vi "PeriodicFilter-Format Stop Filter Entrys.vi"(7 "Seconds Since 1Jan1904 2":timestamp, 10 "Time Format String":string="%<%H:%M:%S%3u>T", 11 "Removed Info":T1[](array[typedef])) -> (3 "Array":string[](array[string]))   [LabVIEW 2017, in "Communicable State Machine.lvlib"]
uses:
  Communicable State Machine.lvlib
  Periodic String Filter Info.ctl
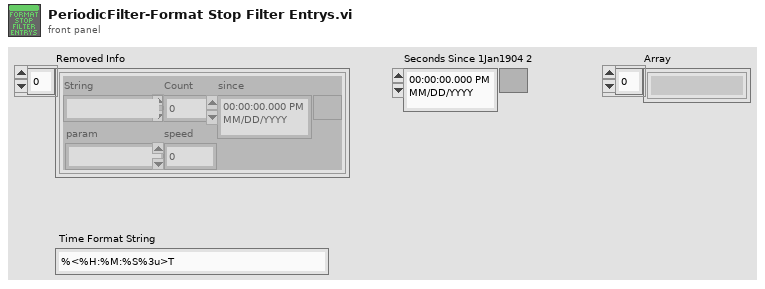
[diagram p1: front panel]
types:
  T1 = typedef "Communicable State Machine.lvlib/Periodic String Filter Info.ctl" = cluster{"String":string, "Count":i64, "since":timestamp, "param":string, "speed":dbl}
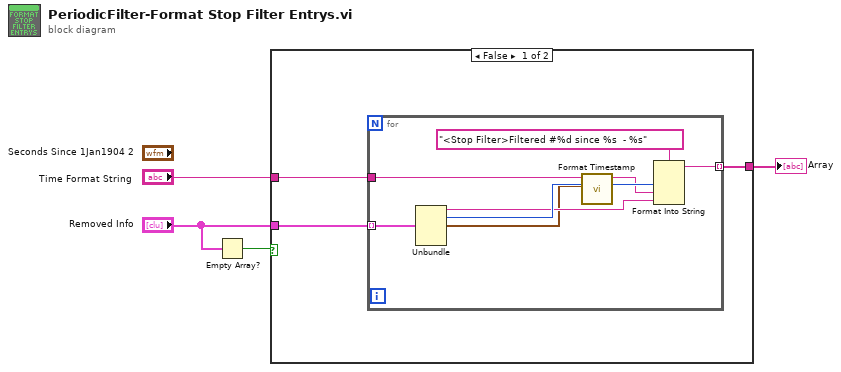
[diagram p0: block diagram]
diagram:
  n1 = Empty Array?(array="Removed Info") -> (empty?=w1:bool)
  n2 = case shown="False" w1 {
    tunnel: "Time Format String" -> [w7 _]
    tunnel: [w6 _] -> w3
    tunnel: "Removed Info" -> [w5 _]
    frame False {
      n3 = for {
        tunnel: w5 -> [w10] mode=indexing
        tunnel: [w9] -> w6 mode=indexing
        tunnel: w7 -> [w8]
        n4 = Unbundle(w10) -> ("String"=w13:string, "Count"=w14:i64, "since"=w12:timestamp)  [unwired: 2 out]
        n5 = call "Format Timestamp.vi"("Timestamp"=w12, "Format String"=w8) -> ("String"=w11:string)  [unwired: 9 in]
        n6 = Format Into String(format string="<Stop Filter>Filtered #%d since %s  - %s", w14, w11, w13) -> (resulting string=w9:string)  [unwired: 2 in, 1 out]
      }
    }
    frame True {
    }
  }
  "Array" <- w3
